vi "set LTE Modulation Index Table Type.vi"(8 "error in (no error)":errorcluster, 9 "256QAM Enable":bool, 10 "64QAM Enable":bool, 11 "Anritsu Call Box_Implement in":refnum<class "Anritsu Call Box_Implement.lvclass">) -> (0 "error out":errorcluster, 3 "Anritsu Call Box_Implement out":refnum<class "Anritsu Call Box_Implement.lvclass">)   [LabVIEW 2023, in "ANRITSU Call Box.lvlib" / "Anritsu Call Box_Implement.lvclass"]
uses:
  Anritsu Call Box_Implement.lvclass
  Anritsu Call Box_Implement.lvclass/Anritsu Call Box_Implement.ctl
  LTE/LTE.lvclass
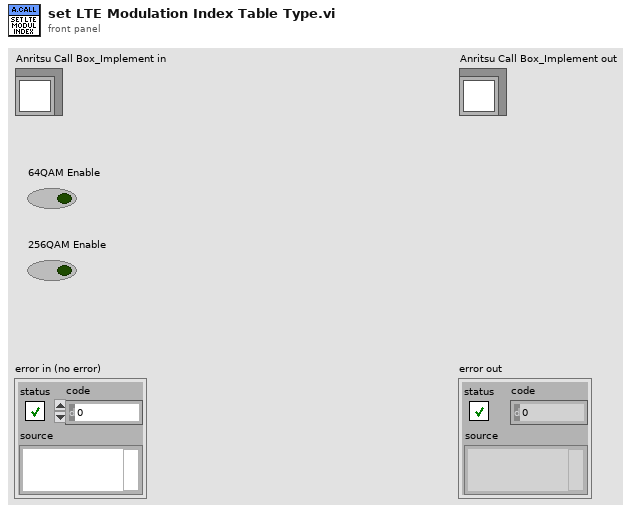
[diagram p1: front panel]
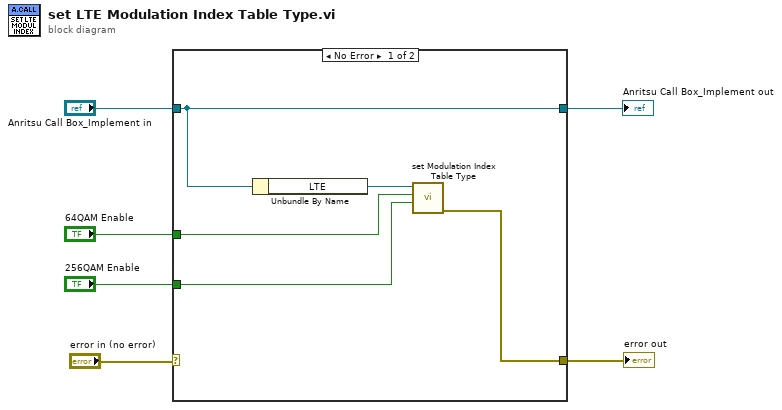
[diagram p0: block diagram]
diagram:
  n1 = case shown="No Error" "error in (no error)" {
    selector: "error in (no error)" -> [_ w12]
    tunnel: "Anritsu Call Box_Implement in" -> [w11 w13]
    tunnel: [w11 w13] -> w5
    tunnel: [w7 w12] -> w3
    tunnel: "64QAM Enable" -> [w9 _]
    tunnel: "256QAM Enable" -> [w8 _]
    frame No Error {
      n2 = Unbundle By Name(w11) -> ("LTE"=w10:refnum<class "LTE.lvclass">)
      n3 = call "set Modulation Index Table Type.vi"("256QAM Enable"=w8, "64QAM Enable"=w9, "LTE in"=w10) -> ("error out"=w7:errorcluster)  [unwired: 7 in, 1 out]
    }
    frame Error {
    }
  }
  "error out" <- w3
  "Anritsu Call Box_Implement out" <- w5
